vi "Read Batch Values - Double.vi"(8 "error in (no error)":errorcluster, 11 "OD Batch in":refnum<class "OD Batch.lvclass">) -> (0 "error out":errorcluster, 2 "Array":dbl[](array[numeric]), 3 "OD Batch out":refnum<class "OD Batch.lvclass">)   [LabVIEW 2023, in "xnet_canopen.lvlib" / "OD Batch.lvclass"]
doc: "Expect OD Vars are all numeric types.\n\nFor I64 and U64, use <b>Type Cast</b> to restore exact value from double; For other types, use directly conversion."
uses:
  OD Batch.lvclass
  OD Batch.lvclass/OD Batch.ctl
  Read Batch OD By Array Index - u64.vi
  Read Batch OD By Array Index - f32.vi
  Read Batch OD By Array Index - u8.vi
  Read Batch OD By Array Index - i8.vi
  Read Batch OD By Array Index - u32.vi
  Read Batch OD By Array Index - f64.vi
  Read Batch OD By Array Index - i32.vi
  Read Batch OD By Array Index - bool.vi
  Read Batch OD By Array Index - u16.vi
  Read Batch OD By Array Index - i64.vi
  Read Batch OD By Array Index - i16.vi
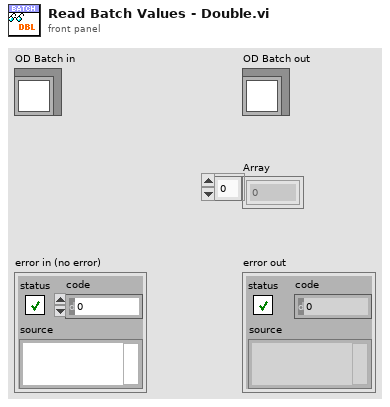
[diagram p1: front panel]
types:
  T1 = typedef "xnet_canopen.lvlib/od entry.ctl" = cluster{"OD Index":T2, "CANOpen Types":T3, "Size":u32, "Offset":u32, "Value":variant, "Initialized":bool}
  T2 = typedef "xnet_canopen.lvlib/od index.ctl" = cluster{"Index":u16, "SubIndex":u8}
  T3 = typedef "xnet_canopen.lvlib/canopen types.ctl" = u32
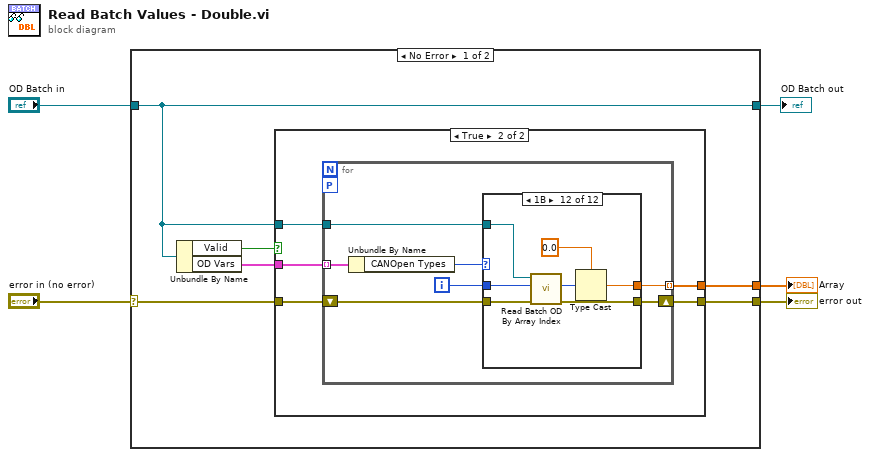
[diagram p0: block diagram]
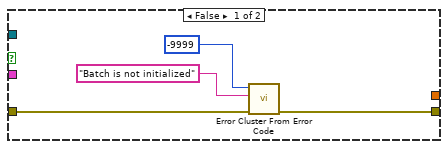
[diagram p2: hidden frame]
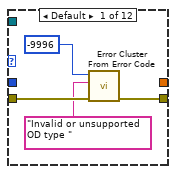
[diagram p3: hidden frame]
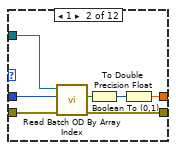
[diagram p4: hidden frame]
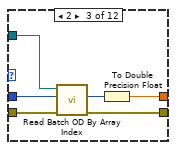
[diagram p5: hidden frame]
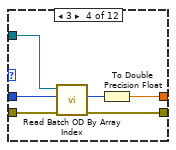
[diagram p6: hidden frame]
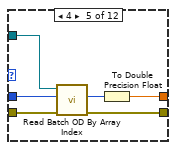
[diagram p7: hidden frame]
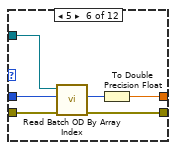
[diagram p8: hidden frame]
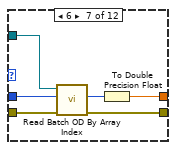
[diagram p9: hidden frame]
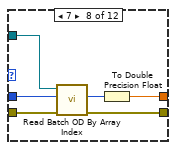
[diagram p10: hidden frame]
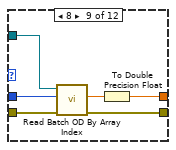
[diagram p11: hidden frame]
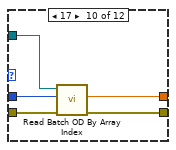
[diagram p12: hidden frame]
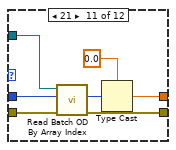
[diagram p13: hidden frame]
diagram:
  n1 = case shown="No Error" "error in (no error)" {
    selector: "error in (no error)" -> [w11 w100]
    tunnel: [w10 w100] -> w4
    tunnel: [w8 w101] -> w2
    tunnel: "OD Batch in" -> [w8 w101]
    tunnel: [w7 _] -> w1
    frame No Error {
      n2 = Unbundle By Name(w8) -> ("Valid"=w6:bool, "OD Vars"=w9:T1[])
      n3 = case shown="True" w6 {
        tunnel: w11 -> [w13 w20]
        tunnel: [w12 w19] -> w10
        tunnel: w9 -> [_ w18]
        tunnel: w8 -> [_ w17]
        tunnel: [_ w16] -> w7
        frame False {
          n4 = call <vilib>:"Error Cluster From Error Code.vi"("error in (no error)"=w13, "error message (\"\")"="Batch is not initialized" ("error message (\"\")"), "error code (0)"=-9999) -> ("error out"=w12:errorcluster)  [unwired: 6 in]
        }
        frame True {
          n5 = for {
            shift-right: [w26] -> w19
            shift-left: w20 -> [w27]
            tunnel: w18 -> [w25] mode=indexing
            workers-P: _ -> [_]
            tunnel: w17 -> [w22]
            tunnel: [w21] -> w16 mode=indexing
            i -> [w23]
            n6 = Unbundle By Name(w25) -> ("CANOpen Types"=w24:T3)
            n7 = case shown="1B" w24 {
              tunnel: w27 -> [w31 w38 w44 w50 w56 w62 w68 w74 w80 w85 w92 w99]
              tunnel: [w30 w37 w43 w49 w55 w61 w67 w73 w79 w84 w91 w98] -> w26
              tunnel: w23 -> [_ w36 w42 w48 w54 w60 w66 w72 w78 w83 w90 w97]
              tunnel: w22 -> [_ w35 w41 w47 w53 w59 w65 w71 w77 w82 w89 w96]
              tunnel: [_ w33 w39 w45 w51 w57 w63 w69 w75 w81 w87 w94] -> w21
              frame Default {
                n8 = call <vilib>:"Error Cluster From Error Code.vi"("error in (no error)"=w31, "error message (\"\")"="Invalid or unsupported OD type " ("error message (\"\")"), "error code (0)"=-9996) -> ("error out"=w30:errorcluster)  [unwired: 6 in]
              }
              frame 1 {
                n9 = call-poly "Read Batch OD By Array Index.vi"("error in (no error)"=w38, "array index"=w36, "OD Batch in"=w35) -> ("error out"=w37:errorcluster, "value"=w34:bool)  [unwired: 6 in, 1 out]
                n10 = Boolean To (0,1)(Boolean=w34) -> (0, 1=w32:i16)
                n11 = To Double Precision Float(number=w32) -> (double precision float=w33:dbl)
              }
              frame 2 {
                n12 = call-poly "Read Batch OD By Array Index.vi"("error in (no error)"=w44, "array index"=w42, "OD Batch in"=w41) -> ("error out"=w43:errorcluster, "value"=w40:i8)  [unwired: 6 in, 1 out]
                n13 = To Double Precision Float(number=w40) -> (double precision float=w39:dbl)
              }
              frame 3 {
                n14 = call-poly "Read Batch OD By Array Index.vi"("error in (no error)"=w50, "array index"=w48, "OD Batch in"=w47) -> ("error out"=w49:errorcluster, "value"=w46:i16)  [unwired: 6 in, 1 out]
                n15 = To Double Precision Float(number=w46) -> (double precision float=w45:dbl)
              }
              frame 4 {
                n16 = call-poly "Read Batch OD By Array Index.vi"("error in (no error)"=w56, "array index"=w54, "OD Batch in"=w53) -> ("error out"=w55:errorcluster, "value"=w52:i32)  [unwired: 6 in, 1 out]
                n17 = To Double Precision Float(number=w52) -> (double precision float=w51:dbl)
              }
              frame 5 {
                n18 = call-poly "Read Batch OD By Array Index.vi"("error in (no error)"=w62, "array index"=w60, "OD Batch in"=w59) -> ("error out"=w61:errorcluster, "value"=w58:u8)  [unwired: 6 in, 1 out]
                n19 = To Double Precision Float(number=w58) -> (double precision float=w57:dbl)
              }
              frame 6 {
                n20 = call-poly "Read Batch OD By Array Index.vi"("error in (no error)"=w68, "array index"=w66, "OD Batch in"=w65) -> ("error out"=w67:errorcluster, "value"=w64:u16)  [unwired: 6 in, 1 out]
                n21 = To Double Precision Float(number=w64) -> (double precision float=w63:dbl)
              }
              frame 7 {
                n22 = call-poly "Read Batch OD By Array Index.vi"("error in (no error)"=w74, "array index"=w72, "OD Batch in"=w71) -> ("error out"=w73:errorcluster, "value"=w70:u32)  [unwired: 6 in, 1 out]
                n23 = To Double Precision Float(number=w70) -> (double precision float=w69:dbl)
              }
              frame 8 {
                n24 = call-poly "Read Batch OD By Array Index.vi"("error in (no error)"=w80, "array index"=w78, "OD Batch in"=w77) -> ("error out"=w79:errorcluster, "value"=w76:sgl)  [unwired: 6 in, 1 out]
                n25 = To Double Precision Float(number=w76) -> (double precision float=w75:dbl)
              }
              frame 17 {
                n26 = call-poly "Read Batch OD By Array Index.vi"("error in (no error)"=w85, "array index"=w83, "OD Batch in"=w82) -> ("error out"=w84:errorcluster, "value"=w81:dbl)  [unwired: 6 in, 1 out]
              }
              frame 21 {
                n27 = call-poly "Read Batch OD By Array Index.vi"("error in (no error)"=w92, "array index"=w90, "OD Batch in"=w89) -> ("error out"=w91:errorcluster, "value"=w88:i64)  [unwired: 6 in, 1 out]
                n28 = Type Cast(type=0.0, x=w88) -> (*(type *) &x=w87:dbl)
              }
              frame 27 {
                n29 = call-poly "Read Batch OD By Array Index.vi"("error in (no error)"=w99, "array index"=w97, "OD Batch in"=w96) -> ("error out"=w98:errorcluster, "value"=w95:u64)  [unwired: 6 in, 1 out]
                n30 = Type Cast(type=0.0, x=w95) -> (*(type *) &x=w94:dbl)
              }
            }
          }
        }
      }
    }
    frame Error {
    }
  }
  "error out" <- w4
  "OD Batch out" <- w2
  "Array" <- w1
